vi "DrawFormattedMultilineString_SubVI.vi"(0 "PictureIn":picture, 1 "FormattedMultiLineStringIn":string="123<B>ABCD</B>456\nAAA<B>BBB<I>CCC<U>DDD</U>EEE</I>FFF</B>GGG\n<I>QWERTY</I>\n<U>D<B>123</B>D</U>E", 2 "TextRectangle":T2={"x"=10.0, "y"=10.0, "width"=150.0, "height"=200.0} {"height" format="%.2f"; "width" format="%.2f"; "y" format="%.2f"; "x" format="%.2f"}, 3 "Justification":T1=enum."RIGHT", 4 "GAP":i32, 5 "Font":T3={"Font Name:"="Arial", "Size"=14, "Strikeout?"=FALSE, "Italic?"=FALSE, "Underline?"=FALSE, "Outline?"=FALSE, "Shadow?"=FALSE, "Bold?"=FALSE}, 6 "scaleY":dbl=2.0, 7 "Color":u32(colorbox), 8 "scaleX":dbl=2.0) -> (14 "PictureOut":picture, 16 "NoChange":bool=TRUE)   [LabVIEW 2020, in "Graphics.lvclass"]
uses:
  <resource>/Framework/Providers/Open_GDS/UML/Graphics_class/Graphics.lvclass
  <resource>/Framework/Providers/Open_GDS/UML/General/Rectangle/Rectangle Rectangle2D.ctl
  <resource>/Framework/Providers/Open_GDS/UML/MultiLineString_class/JustificationType.ctl
  <resource>/Framework/Providers/Open_GDS/UML/MultiLineString_class/MultiLineString.lvclass
panel:
  # "Layout:\nRemove \\r\\n\nSplit in lines-array\nCalc width per char\nGet number of chars to use for line,\nif rest characters, add these to beggining of  lines-array.\nCalc Bound\nAdd \\r\\n where new lines breaks are"
  # "Drawing:\nRemove \\r, split line using \\n\nfor every line calc total length.\n\nFor each line\n  If left start\n  X=B.X+Gap\n  Right:\n  X=B.X+B.W-L.length-Gap\n  Center:\n  X=B.X+(B.W/2)-(L.length/2)\n  Draw Line\nEnd For"
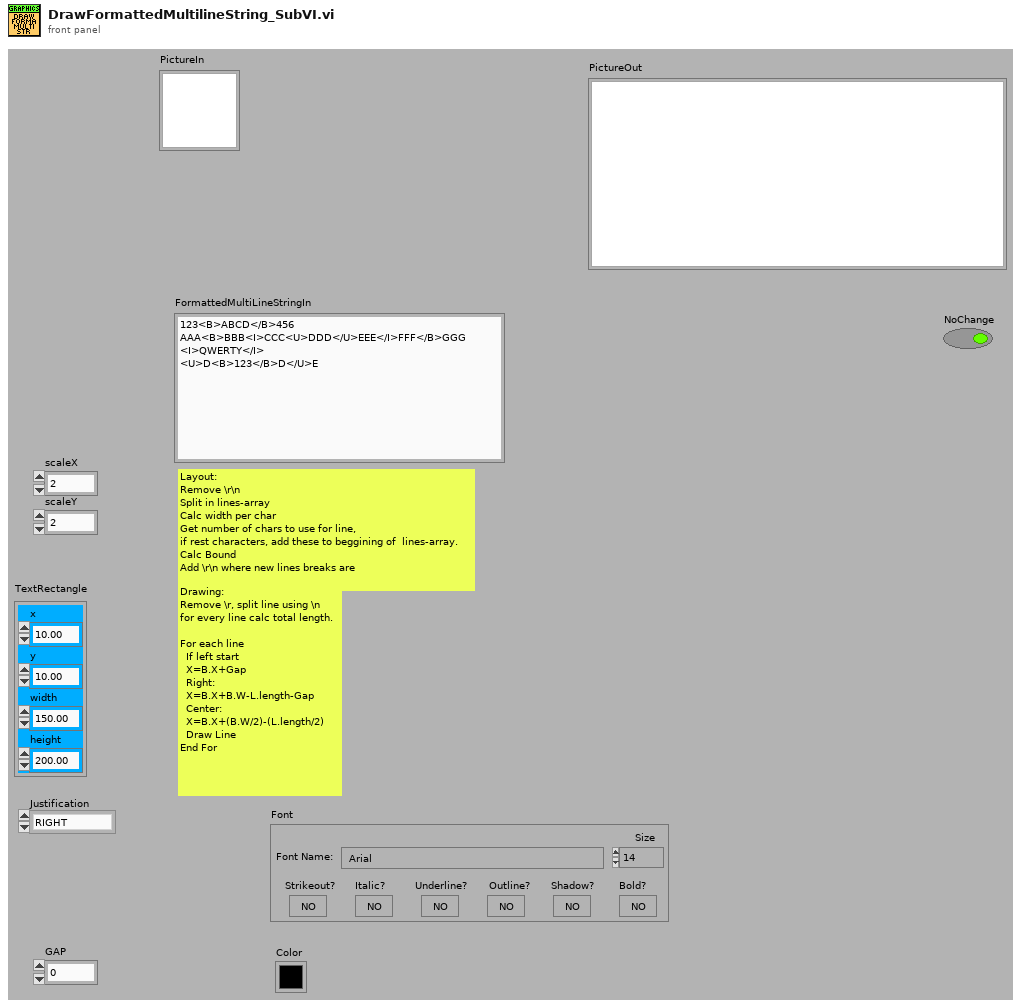
[diagram p1: front panel]
types:
  T1 = typedef "MultiLineString.lvclass/JustificationType.ctl" = enum16{"LEFT", "CENTER", "RIGHT"}
  T2 = typedef "Rectangle Rectangle2D.ctl" = cluster{"x":dbl, "y":dbl, "width":dbl, "height":dbl}
  T3 = cluster{"Font Name:":string, "Size":i16, "Strikeout?":bool, "Italic?":bool, "Underline?":bool, "Outline?":bool, "Shadow?":bool, "Bold?":bool}
  T4 = enum16{"User-specified Font", "Application Font", "System Font", "Dialog Font"}
  T5 = cluster{"horizontal":enum16{"left", "center", "right"}, "vertical":enum16{"top", "center", "bottom"}}
  T6 = cluster{cluster{"Start":i32, "Stop":i32, "Font":cluster{"Font Name:":string, "Size":i16, "Strikeout?":bool, "Italic?":bool, "Underline?":bool, "Outline?":bool, "Shadow?":bool, "Bold?":bool}, "Color":u32}[]}[]
  T7 = cluster{"Start":i32, "Stop":i32, "Font":cluster{"Font Name:":string, "Size":i16, "Strikeout?":bool, "Italic?":bool, "Underline?":bool, "Outline?":bool, "Shadow?":bool, "Bold?":bool}, "Color":u32}[]
  T8 = cluster{"left":i16, "top":i16, "right":i16, "bottom":i16}
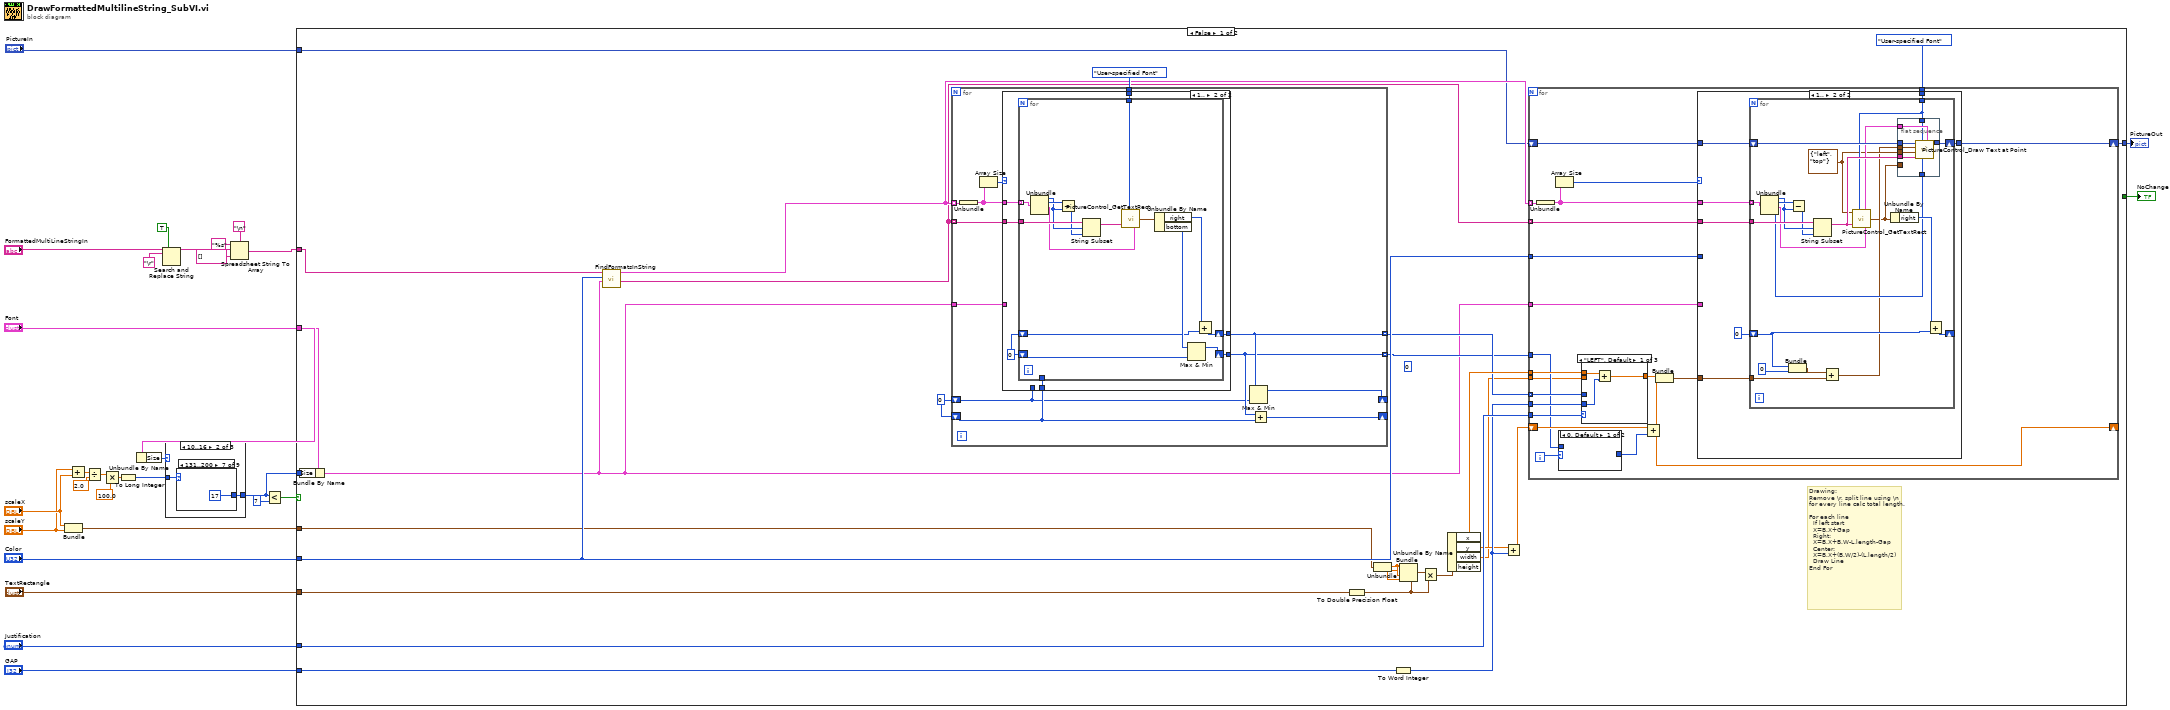
[diagram p0: block diagram]
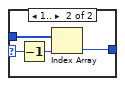
[diagram p2: hidden frame]
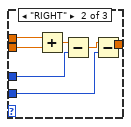
[diagram p3: hidden frame]
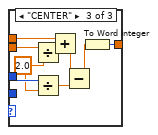
[diagram p4: hidden frame]
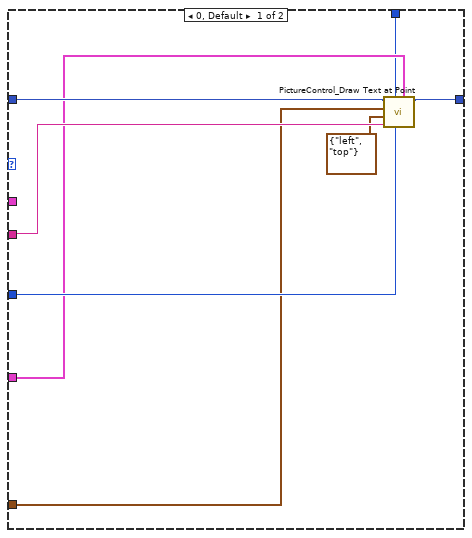
[diagram p5: hidden frame]
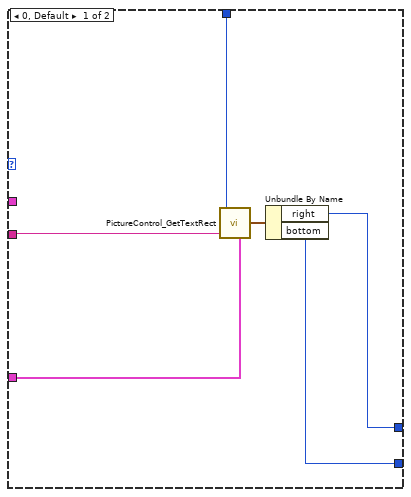
[diagram p6: hidden frame]
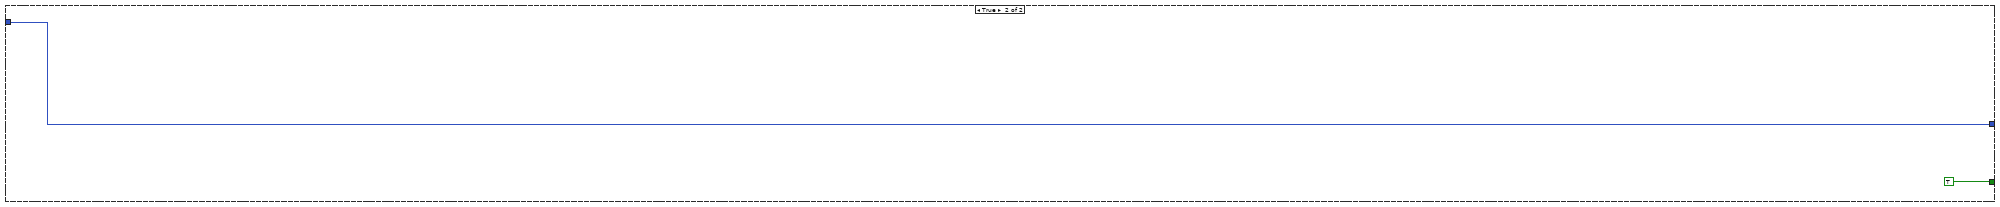
[diagram p7: hidden frame]
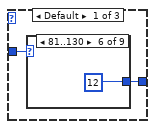
[diagram p8: hidden frame]
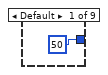
[diagram p9: hidden frame]
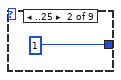
[diagram p10: hidden frame]
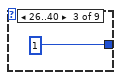
[diagram p11: hidden frame]
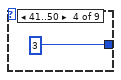
[diagram p12: hidden frame]
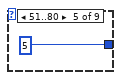
[diagram p13: hidden frame]
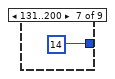
[diagram p14: hidden frame]
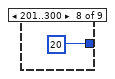
[diagram p15: hidden frame]
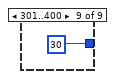
[diagram p16: hidden frame]
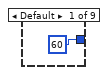
[diagram p17: hidden frame]
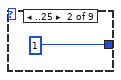
[diagram p18: hidden frame]
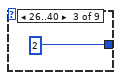
[diagram p19: hidden frame]
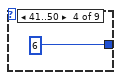
[diagram p20: hidden frame]
diagram:
  n1 = Bundle("scaleX"="scaleX", "scaleY"="scaleY") -> (w2:cluster{"scaleX":dbl, "scaleY":dbl})  [unwired: 1 out]
  n2 = Add(x="scaleY", y="scaleX") -> (x+y=w20:dbl)
  n3 = Divide(x=w20, y=2.0) -> (x/y=w18:dbl)
  n4 = Multiply(x=w18, y=100.0) -> (x*y=w16:dbl)
  n5 = To Long Integer(number=w16) -> (32bit integer=w15:i32)
  n6 = Unbundle By Name("Font") -> ("Size"=w10:i16)
  n7 = Search and Replace String(replace all?=TRUE ("replace all? (F)"), input string="FormattedMultiLineStringIn", search string="\r" ("delimiter (Tab)")) -> (result string=w23:string)  [unwired: 5 in, 3 out]
  n8 = case shown="10..16" w10 {
    tunnel: [w31 w42 w52] -> w9
    tunnel: w15 -> [w30 w41 w53]
    frame Default {
      n9 = case shown="81..130" w30 {
        tunnel: [i16 50 ("Size 9") i16 1 ("Size") i16 1 ("Size 2") i16 3 ("Size 3") i16 5 ("Size 4") i16 12 ("Size 5") i16 14 ("Size 6") i16 20 ("Size 7") i16 30 ("Size 8")] -> w31
        frame Default {
        }
        frame ..25 {
        }
        frame 26..40 {
        }
        frame 41..50 {
        }
        frame 51..80 {
        }
        frame 81..130 {
        }
        frame 131..200 {
        }
        frame 201..300 {
        }
        frame 301..400 {
        }
      }
    }
    frame 10..16 {
      n10 = case shown="131..200" w41 {
        tunnel: [i16 60 ("Size 9") i16 1 ("Size") i16 2 ("Size 2") i16 6 ("Size 3") i16 7 ("Size 4") i16 14 ("Size 5") i16 17 ("Size 6") i16 25 ("Size 7") i16 40 ("Size 8")] -> w42
        frame Default {
        }
        frame ..25 {
        }
        frame 26..40 {
        }
        frame 41..50 {
        }
        frame 51..80 {
        }
        frame 81..130 {
        }
        frame 131..200 {
        }
        frame 201..300 {
        }
        frame 301..400 {
        }
      }
    }
    frame 17.. {
      n11 = case shown="201..300" w53 {
        tunnel: [i16 82 ("Size") i16 2 ("Size") i16 5 ("Size") i16 7 ("Size") i16 12 ("Size") i16 18 ("Size") i16 26 ("Size") i16 36 ("Size") i16 55 ("Size")] -> w52
        frame Default {
        }
        frame ..25 {
        }
        frame 26..40 {
        }
        frame 41..50 {
        }
        frame 51..80 {
        }
        frame 81..130 {
        }
        frame 131..200 {
        }
        frame 201..300 {
        }
        frame 301..400 {
        }
      }
    }
  }
  n12 = Spreadsheet String To Array(delimiter (Tab)="\n", format string="%s", spreadsheet string=w23, array type (2D Dbl)=string[] []) -> (array=w27:string[])
  n13 = Less?(x=w9, y=i16 7) -> (x < y?=w4:bool)
  n14 = case shown="False" w4 {
    tunnel: w27 -> [w90 _]
    tunnel: [w85 w219] -> w22
    tunnel: "TextRectangle" -> [w84 _]
    tunnel: "Color" -> [w83 _]
    tunnel: w9 -> [w82 _]
    tunnel: "Justification" -> [w80 _]
    tunnel: "GAP" -> [w79 _]
    tunnel: "Font" -> [w71 _]
    tunnel: w2 -> [w69 _]
    tunnel: "PictureIn" -> [w64 w219]
    tunnel: [_ TRUE] -> w3
    frame False {
      (unwired) 0 ("index")
      w88 = i16 0
      # "Drawing:\nRemove \\r, split line using \\n\nfor every line calc total length.\n\nFor each line\n  If left start\n  X=B.X+Gap\n  Right:\n  X=B.X+B.W-L.length-Gap\n  Center:\n  X=B.X+(B.W/2)-(L.length/2)\n  Draw Line\nEnd For"
      n15 = Bundle By Name(cluster=w71, "Size"=w82) -> (w63:T3)
      n16 = call <resource>:"FindFormatsInString.vi"("Font"=w63, "Color"=w83, "StringsIn"=w90) -> ("StringsOut"=w86:string[], "Formats"=w87:T6)  [unwired: 7 in]
      n17 = for {
        tunnel: w87 -> [w189] mode=indexing
        tunnel: w86 -> [w188] mode=indexing
        tunnel: T4."User-specified Font" ("desired font(Application)") -> [w187]
        shift-right: [w186] -> _
        shift-left: w88 -> [w179]
        shift-right: [w185] -> _
        shift-left: w88 -> [w178]
        tunnel: [w184] -> w78 mode=indexing
        tunnel: [w183] -> w73 mode=indexing
        tunnel: w63 -> [w180]
        n18 = Unbundle(w189) -> (w182:T7)
        n19 = Array Size(array=w182) -> (size(s)=w181:i32)
        n20 = case shown="1.." w181 {
          tunnel: w188 -> [w191 w202]
          tunnel: w187 -> [w192 w201]
          tunnel: [w193 w199] -> w184
          tunnel: [w194 w198] -> w183
          tunnel: w182 -> [_ w197]
          tunnel: w180 -> [w190 _]
          tunnel: w179 -> [_ w196]
          tunnel: w178 -> [_ _]
          frame 0, Default {
            n21 = call <resource>:"PictureControl_GetTextRect.vi"("desired font(Application)"=w192, "text"=w191, "[user-specified font]"=w190) -> ("rect"=w195:T8)  [unwired: 6 in]
            n22 = Unbundle By Name(w195) -> ("right"=w193:i16, "bottom"=w194:i16)
          }
          frame 1.. {
            w200 = i16 0
            n23 = for {
              tunnel: w202 -> [w216]
              tunnel: w197 -> [w217] mode=indexing
              tunnel: w201 -> [w204]
              shift-right: [w207] -> w199
              shift-left: w200 -> [w205]
              shift-right: [w209] -> w198
              shift-left: w200 -> [w210]
              tunnel: w196 -> [_]
              n24 = Unbundle(w217) -> ("Start"=w214:i32, "Stop"=w215:i32, "Font"=w203:T3)  [unwired: 1 out]
              n25 = Subtract(x=w215, y=w214) -> (x-y=w213:i32)
              n26 = String Subset(string=w216, offset (0)=w214, length (rest)=w213) -> (substring=w206:string)
              n27 = call <resource>:"PictureControl_GetTextRect.vi"("desired font(Application)"=w204, "text"=w206, "[user-specified font]"=w203) -> ("rect"=w212:T8)  [unwired: 6 in]
              n28 = Unbundle By Name(w212) -> ("right"=w208:i16, "bottom"=w211:i16)
              n29 = Max & Min(x=w211, y=w210) -> (max(x,y)=w209:i16)  [unwired: 1 out]
              n30 = Add(x=w208, y=w205) -> (x+y=w207:i16)
            }
          }
        }
        n31 = Max & Min(x=w184, y=w178) -> (max(x,y)=w185:i16)  [unwired: 1 out]
        n32 = Add(x=w183, y=w179) -> (x+y=w186:i16)
      }
      n33 = To Double Precision Float(number=w84) -> (double precision float=w66:T2)
      n34 = Unbundle(w69) -> ("scaleX"=w68:dbl, "scaleY"=w67:dbl)
      n35 = To Word Integer(number=w79) -> (16bit integer=w77:i16)
      n36 = Bundle(cluster=w66, "x"=w68, "y"=w67, "width"=w68, "height"=w67) -> (w65:T2)
      n37 = Multiply(x=w65, y=w66) -> (x*y=w70:T2)
      n38 = Unbundle By Name(w70) -> ("x"=w81:dbl, "y"=w76:dbl, "width"=w72:dbl)  [unwired: 1 out]
      n39 = Add(x=w76, y=w77) -> (x+y=w75:dbl)
      n40 = for {
        tunnel: w87 -> [w111] mode=indexing
        tunnel: w86 -> [w110] mode=indexing
        tunnel: w63 -> [w107]
        shift-right: [w105] -> w85
        shift-left: w64 -> [w106]
        tunnel: w83 -> [w104]
        tunnel: w81 -> [w98]
        tunnel: w80 -> [w99]
        tunnel: w77 -> [w101]
        tunnel: w78 -> [w100] mode=indexing
        tunnel: w73 -> [w94]
        shift-right: [w96] -> _
        shift-left: w75 -> [w102]
        tunnel: T4."User-specified Font" ("desired font(Application)") -> [w95]
        tunnel: w72 -> [w91]
        i -> [w92]
        n41 = Unbundle(w111) -> (w109:T7)
        n42 = Array Size(array=w109) -> (size(s)=w108:i32)
        n43 = case shown="0, Default" w92 {
          selector: w92 -> [_ w112]
          tunnel: w94 -> [_ w115]
          tunnel: [_ w113] -> w93
          frame 0, Default {
          }
          frame 1.. {
            n44 = Decrement(x=w112) -> (x-1=w114:i32)
            n45 = Index Array(array=w115, index=w114) -> (element=w113:i16)
          }
        }
        n46 = case shown="\"LEFT\", Default" w99 {
          tunnel: w100 -> [_ w121 w128]
          tunnel: w98 -> [w118 w119 w133]
          tunnel: w101 -> [w117 w125 _]
          tunnel: [w116 w124 w132] -> w103
          tunnel: w91 -> [_ w120 w131]
          frame "LEFT", Default {
            n47 = Add(x=w118, y=w117) -> (x+y=w116:dbl)
          }
          frame "RIGHT" {
            n48 = Add(x=w119, y=w120) -> (x+y=w123:dbl)
            n49 = Subtract(x=w123, y=w121) -> (x-y=w122:dbl)
            n50 = Subtract(x=w122, y=w125) -> (x-y=w124:dbl)
          }
          frame "CENTER" {
            w127 = 2.0 ("y")
            n51 = Divide(x=w131, y=w127) -> (x/y=w134:dbl)
            n52 = Divide(x=w128, y=w127) -> (x/y=w126:dbl)
            n53 = Add(x=w133, y=w134) -> (x+y=w130:dbl)
            n54 = Subtract(x=w130, y=w126) -> (x-y=w129:dbl)
            n55 = To Word Integer(number=w129) -> (16bit integer=w132:i16)
          }
        }
        n56 = Add(x=w102, y=w93) -> (x+y=w96:dbl)
        n57 = Bundle(w103, w96) -> (w97:cluster{dbl, dbl})  [unwired: 1 in]
        n58 = case shown="1.." w108 {
          tunnel: w110 -> [w140 w149]
          tunnel: w109 -> [_ w147]
          tunnel: w107 -> [w137 _]
          tunnel: w106 -> [w142 w146]
          tunnel: [w141 w145] -> w105
          tunnel: w104 -> [w138 _]
          tunnel: w97 -> [w135 w143]
          tunnel: w95 -> [w136 w144]
          frame 0, Default {
            n59 = call <resource>:"PictureControl_Draw Text at Point.vi"("[user-specified font]"=w137, "text color(black)"=w138, "desired font(Application)"=w136, "text"=w140, "alignment(left, top)"=T5 {"horizontal"=enum."left", "vertical"=enum."top"}, "origin"=w135, "picture"=w142) -> ("new picture"=w141:picture)  [unwired: 3 in, 1 out]
          }
          frame 1.. {
            n60 = for {
              tunnel: w149 -> [w168]
              tunnel: w147 -> [w169] mode=indexing
              shift-right: [w163] -> _
              shift-left: i16 0 -> [w159]
              shift-right: [w161] -> w145
              shift-left: w146 -> [w162]
              tunnel: w143 -> [w156]
              tunnel: w144 -> [w153]
              w152 = T5 {"horizontal"=enum."left", "vertical"=enum."top"} ("alignment(left, top)")
              n61 = Unbundle(w169) -> ("Start"=w166:i32, "Stop"=w167:i32, "Font"=w157:T3, "Color"=w158:u32)
              n62 = Bundle(w159, i16 0) -> (w155:cluster{i16, i16})  [unwired: 1 in]
              n63 = Subtract(x=w167, y=w166) -> (x-y=w165:i32)
              n64 = String Subset(string=w168, offset (0)=w166, length (rest)=w165) -> (substring=w160:string)
              n65 = Add(x=w155, y=w156) -> (x+y=w151:cluster{dbl, dbl})
              n66 = call <resource>:"PictureControl_GetTextRect.vi"("alignment(left, top)"=w152, "desired font(Application)"=w153, "text"=w160, "[user-specified font]"=w157) -> ("rect"=w150:T8)  [unwired: 5 in]
              n67 = Unbundle By Name(w150) -> ("right"=w164:i16)
              n68 = flat-sequence {
                tunnel: w162 -> [w177]
                tunnel: [w176] -> w161
                tunnel: w160 -> [w175]
                tunnel: w158 -> [w174]
                tunnel: w157 -> [w173]
                tunnel: w153 -> [w172]
                tunnel: w152 -> [w171]
                tunnel: w151 -> [w170]
                tunnel: w150 -> [_]
                frame #0 {
                  n69 = call <resource>:"PictureControl_Draw Text at Point.vi"("[user-specified font]"=w173, "text color(black)"=w174, "desired font(Application)"=w172, "text"=w175, "alignment(left, top)"=w171, "origin"=w170, "picture"=w177) -> ("new picture"=w176:picture)  [unwired: 3 in, 1 out]
                }
              }
              n70 = Add(x=w164, y=w159) -> (x+y=w163:i16)
            }
          }
        }
      }
    }
    frame True {
    }
  }
  "PictureOut" <- w22
  "NoChange" <- w3
